vi "FuncVI-viCtrlGet.vi"(5 "InstanceRef":T2, 9 "arg list":T1[](array[typedef]) {"num" format="%.2f"}) -> (0 "error out":bool, 3 "result":T1 {"num" format="%.2f"})   [LabVIEW 2021]
doc: "::: CalcExpress Toolkit :::\nCopyright (c) 2000-2026 Konstantin Shifershteyn. All rights reserved."
uses:
  cetypes.llb/CalcExpress Function Argument Info.ctl
  cetypes.llb/CalcExpress Instance RefNum.ctl
  <vilib>/Utility/error.llb/DialogType.ctl
panel:
  in  "max arg num":i32=1000
  in  "min arg num":i32=3
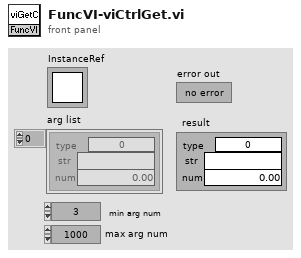
[diagram p1: front panel]
types:
  T1 = typedef "CalcExpress Function Argument Info.ctl" = cluster{"type":u32, "str":string, "num":dbl}
  T2 = typedef "CalcExpress Instance RefNum.ctl" = refnum<k1>
  T3 = cluster{"index":i32, "data type":enum32{"String", "DBL Number", "identifier", "1D Array of DBL", "2D Array of DBL", "CDB Number", "1D Array of CDB", "2D Array of CDB", "1D Array of String", "2D Array of String", "Unknown data type"}, "default num":dbl, "default str":string}[]
  T4 = enum32{"String", "DBL Number", "identifier", "1D Array of DBL", "2D Array of DBL", "CDB Number", "1D Array of CDB", "2D Array of CDB", "1D Array of String", "2D Array of String", "Unknown data type"}
  T5 = typedef "VarMan Variable Context Handle.ctl" = i32
  T6 = cluster{"index":i32, "type":i32, "default num":dbl, "default str":string}[]
  T7 = typedef "DialogType.ctl" = u16
  T8 = typedef "CalcExpress Data Type.ctl" = enum32{"String", "DBL Number", "identifier", "1D Array of DBL", "2D Array of DBL", "CDB Number", "1D Array of CDB", "2D Array of CDB", "1D Array of String", "2D Array of String", "Unknown data type"}
  T9 = cluster{"use this constant to specify a predefined type":enum32{"String", "DBL Number", "identifier", "1D Array of DBL", "2D Array of DBL", "CDB Number", "1D Array of CDB", "2D Array of CDB", "1D Array of String", "2D Array of String", "Unknown data type"}, string, "code":i32}
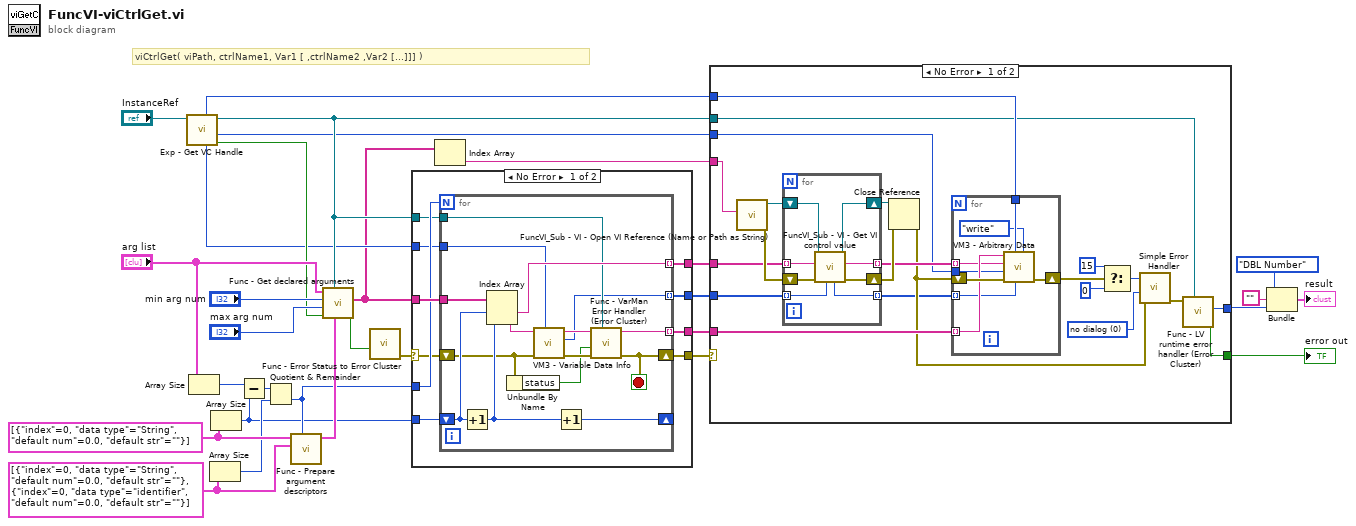
[diagram p0: block diagram]
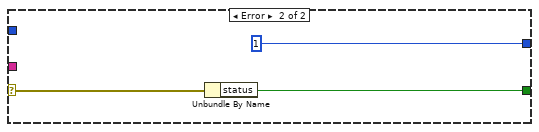
[diagram p2: hidden frame]
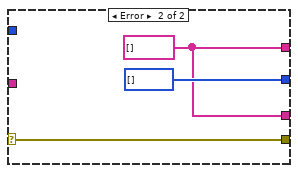
[diagram p3: hidden frame]
diagram:
  w18 = T3 [{"index"=0, "data type"=enum."String", "default num"=0.0, "default str"=""}] ("args descriptors")
  w16 = T3 [{"index"=0, "data type"=enum."String", "default num"=0.0, "default str"=""}, {"index"=0, "data type"=enum."identifier", "default num"=0.0, "default str"=""}] ("args descriptors")
  # "viCtrlGet( viPath, ctrlName1, Var1 [ ,ctrlName2 ,Var2 [...]]] )"
  n1 = call "Exp - Get VC Handle.vi"("InstanceRef"="InstanceRef") -> ("error out"=w9:bool, "writer ID"=w3:u32, "dup InstanceRef"=w11:T2, "VC Handle"=w8:T5)  [unwired: 5 in]
  n2 = Array Size(array="arg list") -> (size(s)=w14:i32)
  n3 = Array Size(array=w16) -> (size(s)=w17:i32)
  n4 = Array Size(array=w18) -> (size(s)=w13:i32)
  n5 = Subtract(x=w14, y=w13) -> (x-y=w15:i32)
  n6 = Quotient & Remainder(x=w15, y=w17) -> (floor(x/y)=w19:i32)  [unwired: 1 out]
  n7 = call "Func - Prepare argument descriptors.vi"("number"=w19, "arg templates"=w16, "arg descriptors in"=w18) -> ("arg descriptors out"=w20:T6)  [unwired: 5 in, 1 out]
  n8 = call "Func - Get declared arguments.vi"("arg descriptors"=w20, "InstanceRef"=w11, "error in"=w9, "max arg num"="max arg num", "min arg num"="min arg num", "arg list"="arg list") -> ("error out"=w1:bool, "str list"=w7:string[])  [unwired: 2 in, 2 out]
  n9 = call "Func - Error Status to Error Cluster.vi"("error status in"=w1) -> ("Error Cluster out"=w2:errorcluster)  [unwired: 9 in, 1 out]
  n10 = case shown="No Error" w2 {
    selector: w2 -> [w35 w57]
    tunnel: [w38 w57] -> w27
    tunnel: w7 -> [w39 _]
    tunnel: [w37 u32[] []] -> w26
    tunnel: w11 -> [w32 _]
    tunnel: w19 -> [w36 _]
    tunnel: w13 -> [w34 _]
    tunnel: [w33 w55] -> w12
    tunnel: w8 -> [w31 _]
    tunnel: [w30 w55] -> w5
    frame No Error {
      n11 = for {
        N: w36 -> [_]
        shift-right: [w54] -> _
        shift-left: w34 -> [w53]
        shift-right: [w43] -> w38
        shift-left: w35 -> [w42]
        tunnel: w39 -> [w52]
        tunnel: [w40] -> w37 mode=indexing
        tunnel: w32 -> [w46]
        tunnel: [w51] -> w33 mode=indexing
        tunnel: w31 -> [w45]
        tunnel: [w44] -> w30 mode=indexing
        stop <- w43 stop-if-true
        n12 = Increment(x=w53) -> (x+1=w50:i32)
        n13 = Index Array(array=w52, index #1=w53, index #2=w50) -> (element #1=w51:string, element #2=w47:string)
        n14 = Unbundle By Name(w42) -> ("status"=w41:bool)
        n15 = call "VM3 - Variable Data Info.vi"("VC Handle"=w45, "error in"=w42, "name_spec"=w47) -> ("error out"=w49:errorcluster, "var type"=w40:u32, "dup name_spec"=w48:string)  [unwired: 3 in, 3 out]
        n16 = Increment(x=w50) -> (x+1=w54:i32)
        n17 = call "Func - VarMan Error Handler (Error Cluster).vi"("InstanceRef"=w46, "VarMan VI error in"=w49, "error status before"=w41, "var name"=w48) -> ("error out"=w43:errorcluster, "dup var name"=w44:string)  [unwired: 5 in, 1 out]
      }
    }
    frame Error {
      w55 = string[] []
    }
  }
  n18 = Index Array(array=w7) -> (element=w4:string)  [unwired: 1 in]
  n19 = case shown="No Error" w27 {
    selector: w27 -> [_ w98]
    tunnel: w26 -> [w79 _]
    tunnel: w4 -> [w76 _]
    tunnel: [w63 w96] -> w6
    tunnel: w11 -> [w65 _]
    tunnel: [w64 1 ("code")] -> w23
    tunnel: w12 -> [w73 _]
    tunnel: w8 -> [w71 _]
    tunnel: w5 -> [w67 _]
    tunnel: w3 -> [w58 _]
    frame No Error {
      w60 = T7 0 items=["no dialog", "OK message", "continue or stop message", "OK message + warnings", "continue/stop + warnings"] ("type of dialog (OK msg:1)")
      n20 = call "FuncVI_Sub - VI - Open VI Reference (Name or Path as String).vi"("VI name or path"=w76) -> ("error out"=w77:errorcluster, "VI Refnum"=w78:refnum<vi>)  [unwired: 9 in]
      n21 = for {
        tunnel: w79 -> [w90] mode=indexing
        shift-right: [w94] -> w74
        shift-left: w77 -> [w95]
        shift-right: [w93] -> w75
        shift-left: w78 -> [w92]
        tunnel: w73 -> [w91] mode=indexing
        tunnel: [w89] -> w72 mode=indexing
        tunnel: [w88] -> w61 mode=indexing
        n22 = call "FuncVI_Sub - VI - Get VI control value.vi"("expected type"=w90, "error in"=w95, "control name"=w91, "VI Ref"=w92) -> ("error out"=w94:errorcluster, "str"=w89:string, "dup VI Ref"=w93:refnum<vi>, "type"=w88:T8)  [unwired: 2 in]
      }
      n23 = Close Reference(reference=w75, error in (no error)=w74) -> (error out=w62:errorcluster)
      n24 = for {
        shift-right: [w86] -> w59
        shift-left: w62 -> [w87]
        tunnel: w72 -> [w83] mode=indexing
        tunnel: w67 -> [w85] mode=indexing
        tunnel: w71 -> [w84]
        tunnel: w61 -> [w82] mode=indexing
        tunnel: w58 -> [w80]
        n25 = call "VM3 - Arbitrary Data.vi"("cmd (read)"=enum16{"create", "destroy", "write", "read"}."write", "var type in"=w82, "VC Handle"=w84, "error in"=w87, "writer ID"=w80, "flattened value in"=w83, "name_spec"=w85) -> ("error out"=w86:errorcluster)  [unwired: 4 out]
      }
      n26 = Select(t=15, s=w59, f=0) -> (s? t:f=w68:i32)
      n27 = call <vilib>:"Simple Error Handler.vi"("error code (no error:0)"=w68, "type of dialog (OK msg:1)"=w60, "error in (no error)"=w62) -> ("error out"=w66:errorcluster)  [unwired: 2 in, 4 out]
      n28 = call "Func - LV runtime error handler (Error Cluster).vi"("InstanceRef"=w65, "LabVIEW error"=w66) -> ("error out"=w63:bool, "LV error code"=w64:i32)  [unwired: 4 in, 2 out]
    }
    frame Error {
      n29 = Unbundle By Name(w98) -> ("status"=w96:bool)
    }
  }
  "error out" <- w6
  n30 = Bundle("use this constant to specify a predefined type"=T4."DBL Number", "", "code"=w23) -> (→"result":T9)  [unwired: 1 in]
